vi "Simple Server.vi"() -> ()   [LabVIEW 2020]
uses:
  source/Server/Server/Server.lvclass
  source/Server/Server/Post - DBL.vi
  source/Server/Server/Add PV - DBL.vi
  source/Server/Server/Fetch - DBL.vi
panel:
  in  "PV name":string="DEV:FLOAT64"
  out "timestamp":timestamp
  in  "Value":dbl format="%.3f"
  in  "Increment":bool
  in  "stop":bool
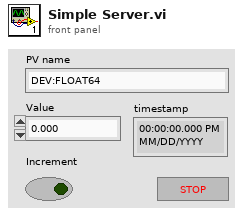
[diagram p1: front panel]
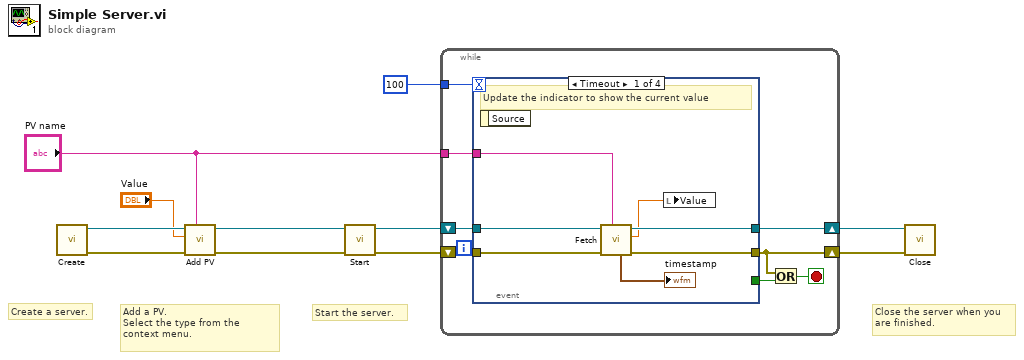
[diagram p0: block diagram]
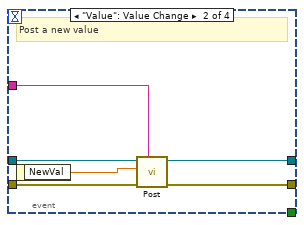
[diagram p2: hidden frame]
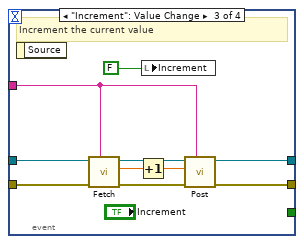
[diagram p3: hidden frame]
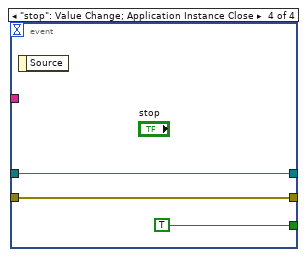
[diagram p4: hidden frame]
diagram:
  # "Close the server when you are finished."
  # "Start the server."
  # "Add a PV.\nSelect the type from the context menu."
  # "Create a server."
  n1 = call "Create.vi"() -> ("error out"=w2:errorcluster, "Server out"=w8:refnum<class "Server.lvclass">)  [unwired: 10 in]
  n2 = call-poly "Add PV.vi"("PV name"="PV name", "error in (no error)"=w2, "initial value"="Value", "Server in"=w8) -> ("error out"=w6:errorcluster, "Server out"=w5:refnum<class "Server.lvclass">)  [unwired: 6 in]
  n3 = call-dynamic "Start.vi"("error in (no error)"=w6, "Server in"=w5) -> ("error out"=w3:errorcluster, "Server out"=w4:refnum<class "Server.lvclass">)  [unwired: 8 in]
  n4 = while {
    tunnel: "PV name" -> [w18]
    shift-right: [w16] -> w9
    shift-left: w4 -> [w17]
    shift-right: [w13] -> w10
    shift-left: w3 -> [w19]
    tunnel: 100 ("Numeric") -> [w12]
    stop <- w14 stop-if-true
    n5 = event shown="[0] Timeout" {
      selector: _ -> [_ _ _ _]
      dyn-events: _ -> [_ _ _ _]
      timeout: w12 -> [_ _ _ _]
      tunnel: w19 -> [w26 w32 w42 w44]
      tunnel: w18 -> [w22 w31 w35 _]
      tunnel: w17 -> [w25 w30 w41 w43]
      tunnel: [w23 w28 w33 w44] -> w13
      tunnel: [w24 w29 w34 w43] -> w16
      tunnel: [_ _ _ TRUE] -> w15
      event Timeout {
        # "Update the indicator to show the current value"
        n6 = event-data() -> ()  [unwired: 1 in, 1 out]
        n7 = call-poly "Fetch.vi"("PV name"=w22, "error in"=w26, "Server in"=w25) -> ("error out"=w23:errorcluster, "value"=w21:dbl, "Server out"=w24:refnum<class "Server.lvclass">, "timestamp"=→"timestamp":timestamp)  [unwired: 4 in, 1 out]
        n8 = local write "Value"(w21) -> ()
      }
      event "Value": Value Change {
        # "Post a new value"
        n9 = event-data() -> ("NewVal"=w27:dbl)  [unwired: 1 in]
        n10 = call-poly "Post.vi"("PV name"=w31, "error in (no error)"=w32, "value"=w27, "Server in"=w30) -> ("error out"=w28:errorcluster, "Server out"=w29:refnum<class "Server.lvclass">)  [unwired: 6 in]
      }
      event "Increment": Value Change {
        # "Increment the current value"
        n11 = event-data() -> ()  [unwired: 1 in, 1 out]
        n12 = call-poly "Fetch.vi"("PV name"=w35, "error in"=w42, "Server in"=w41) -> ("error out"=w38:errorcluster, "value"=w39:dbl, "Server out"=w36:refnum<class "Server.lvclass">)  [unwired: 4 in, 2 out]
        n13 = Increment(x=w39) -> (x+1=w37:dbl)
        n14 = local write "Increment"(FALSE ("Increment")) -> ()
        n15 = call-poly "Post.vi"("PV name"=w35, "error in (no error)"=w38, "value"=w37, "Server in"=w36) -> ("error out"=w33:errorcluster, "Server out"=w34:refnum<class "Server.lvclass">)  [unwired: 6 in]
      }
      event "stop": Value Change; Application Instance Close {
        n16 = event-data() -> ()  [unwired: 1 in, 1 out]
      }
    }
    n17 = Or(x=w13, y=w15) -> (x .or. y?=w14:bool)
  }
  n18 = call-dynamic "Close.vi"("error in"=w10, "Server in"=w9) -> ()  [unwired: 9 in, 1 out]
